vi "Parse LTE Handover Param (L).vi"(8 "error in (no error)":errorcluster caption="에러 입력(에러 없음)", 10 "JSON string":string, 11 "Instrument Manager 입력":refnum<class "Instrument Manager.lvclass">) -> (0 "error out":errorcluster caption="에러 출력", 1 "LTE Call Handover Param":T1, 2 "Call Process Param LTE":T3, 3 "Instrument Manager 출력":refnum<class "Instrument Manager.lvclass">)   [LabVIEW 2023, in "Instrument Manager.lvclass"]
uses:
  Instrument Manager.lvclass
  Instrument Manager.lvclass/Instrument Manager.ctl
  Handover Param LTE.ctl
  Module/ANRITSU Call Box/Type Definition/LTE Supported BandWidth.ctl
  Module/ANRITSU Call Box/ANRITSU Call Box.lvlib
  Type Definition/LTE Handover Param.ctl
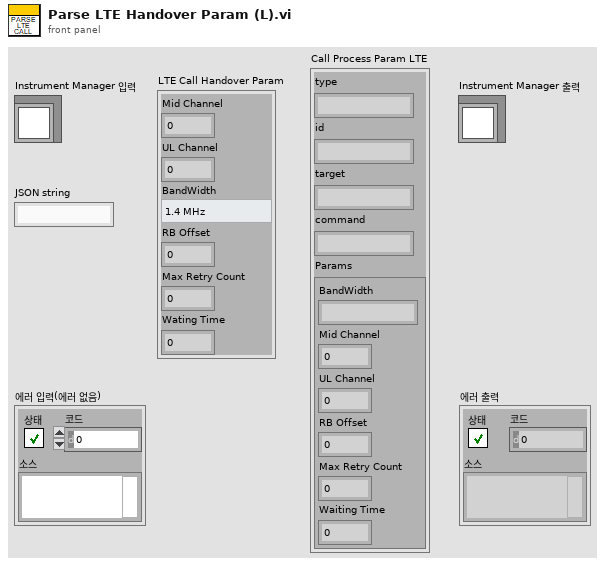
[diagram p1: front panel]
types:
  T1 = typedef "LTE Handover Param.ctl" = cluster{"Mid Channel":i32, "UL Channel":i32, "BandWidth":T2, "RB Offset":i32, "Max Retry Count":i32, "Wating Time":i32}
  T2 = typedef "ANRITSU Call Box.lvlib/LTE Supported BandWidth.ctl" = enum16{"1.4 MHz", "3 MHz", "5 MHz", "10 MHz", "15 MHz", "20 MHz"}
  T3 = typedef "Instrument Manager.lvclass/Handover Param LTE.ctl" = cluster{"type":string, "id":string, "target":string, "command":string, "Params":cluster{"BandWidth":string, "Mid Channel":i32, "UL Channel":i32, "RB Offset":i32, "Max Retry Count":i32, "Waiting Time":i32}}
  T4 = cluster{"BandWidth":string, "Mid Channel":i32, "UL Channel":i32, "RB Offset":i32, "Max Retry Count":i32, "Waiting Time":i32}
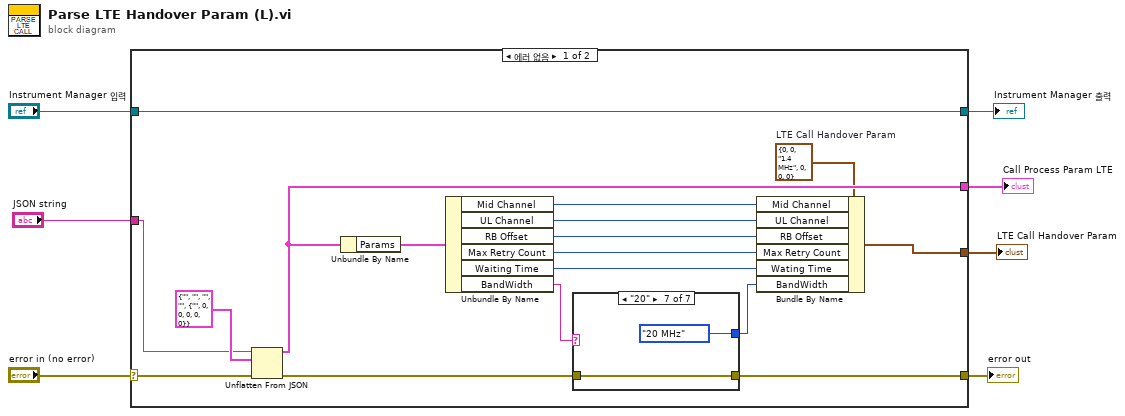
[diagram p0: block diagram]
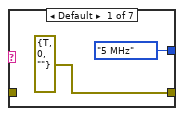
[diagram p2: hidden frame]
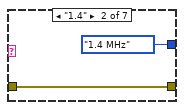
[diagram p3: hidden frame]
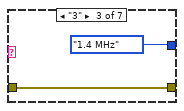
[diagram p4: hidden frame]
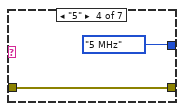
[diagram p5: hidden frame]
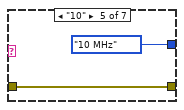
[diagram p6: hidden frame]
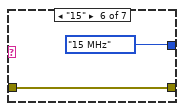
[diagram p7: hidden frame]
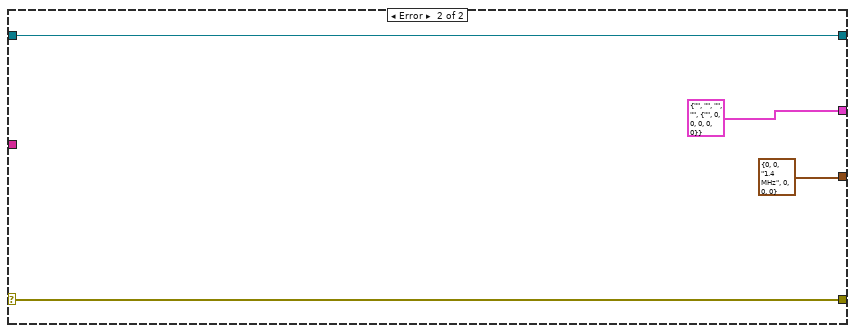
[diagram p8: hidden frame]
diagram:
  n1 = case shown="에러 없음" "error in (no error)" {
    selector: "error in (no error)" -> [w22 w42]
    tunnel: [w10 w42] -> w6
    tunnel: [w24 w41] -> w4
    tunnel: "Instrument Manager 입력" -> [w24 w41]
    tunnel: "JSON string" -> [w21 _]
    tunnel: [w20 T3 {"type"="", "id"="", "target"="", "command"="", "Params"={"BandWidth"="", "Mid Channel"=0, "UL Channel"=0, "RB Offset"=0, "Max Retry Count"=0, "Waiting Time"=0}} ("Call Process Param LTE")] -> w2
    tunnel: [w9 T1 {"Mid Channel"=0, "UL Channel"=0, "BandWidth"=enum."1.4 MHz", "RB Offset"=0, "Max Retry Count"=0, "Wating Time"=0} ("LTE Call Handover Param")] -> w1
    frame No Error {
      w11 = T1 {"Mid Channel"=0, "UL Channel"=0, "BandWidth"=enum."1.4 MHz", "RB Offset"=0, "Max Retry Count"=0, "Wating Time"=0}  # LTE Call Handover Param
      n2 = Unflatten From JSON(JSON string=w21, type and defaults=T3 {"type"="", "id"="", "target"="", "command"="", "Params"={"BandWidth"="", "Mid Channel"=0, "UL Channel"=0, "RB Offset"=0, "Max Retry Count"=0, "Waiting Time"=0}} ("Call Process Param LTE"), error in (no error)=w22) -> (value=w20:T3, error out=w12:errorcluster)  [unwired: 4 in]
      n3 = Unbundle By Name(w20) -> ("Params"=w13:T4)
      n4 = Unbundle By Name(w13) -> ("Mid Channel"=w8:i32, "UL Channel"=w17:i32, "RB Offset"=w16:i32, "Max Retry Count"=w15:i32, "Waiting Time"=w14:i32, "BandWidth"=w19:string)
      n5 = case shown="\"20\"" w19 {
        tunnel: w12 -> [_ w28 w30 w32 w33 w35 w37]
        tunnel: [errorcluster {"status"=TRUE, "code"=0, "source"=""} ("error out") w28 w30 w32 w33 w35 w37] -> w10
        tunnel: [LTE_Supported_BandWidth."5 MHz" ("BandWidth") LTE_Supported_BandWidth."1.4 MHz" ("BandWidth") LTE_Supported_BandWidth."1.4 MHz" ("BandWidth") LTE_Supported_BandWidth."5 MHz" ("BandWidth") LTE_Supported_BandWidth."10 MHz" ("BandWidth") LTE_Supported_BandWidth."15 MHz" ("BandWidth") LTE_Supported_BandWidth."20 MHz" ("BandWidth")] -> w18
        frame Default {
        }
        frame "1.4" {
        }
        frame "3" {
        }
        frame "5" {
        }
        frame "10" {
        }
        frame "15" {
        }
        frame "20" {
        }
      }
      n6 = Bundle By Name(cluster=w11, "Mid Channel"=w8, "UL Channel"=w17, "RB Offset"=w16, "Max Retry Count"=w15, "Wating Time"=w14, "BandWidth"=w18) -> (w9:T1)
    }
    frame Error {
    }
  }
  "error out" <- w6
  "Instrument Manager 출력" <- w4
  "Call Process Param LTE" <- w2
  "LTE Call Handover Param" <- w1
